vi "Create Channel.vi"(8 "error in (no error)":errorcluster, 10 "AIO_CFG":refnum<class "AIO-Configuration.lvclass">, 11 "UI Template in":refnum<class "AIO_Panel.lvclass">) -> (0 "error out":errorcluster, 3 "UI Template out":refnum<class "AIO_Panel.lvclass">)   [LabVIEW 2021, in "Simulator-Channel.lvlib" / "AIO_Panel.lvlib" / "AIO_Panel.lvclass"]
uses:
  AIO_Panel.lvclass
  Dependencies/AIO-Channel.lvlibp/Channels/AIO-Channel/AIO-Configuration_class/AIO-Configuration.lvclass
  C:/Users/averna/Documents/LV Gym DEMO/Factory Pattern/Device Channels/Dependencies/AIO-Channel.lvlibp/Generic Channel/Channel/Configuration_class/Configuration.lvclass
  tdef/info.ctl
  AIO_Panel.lvclass/AIO_Panel.ctl
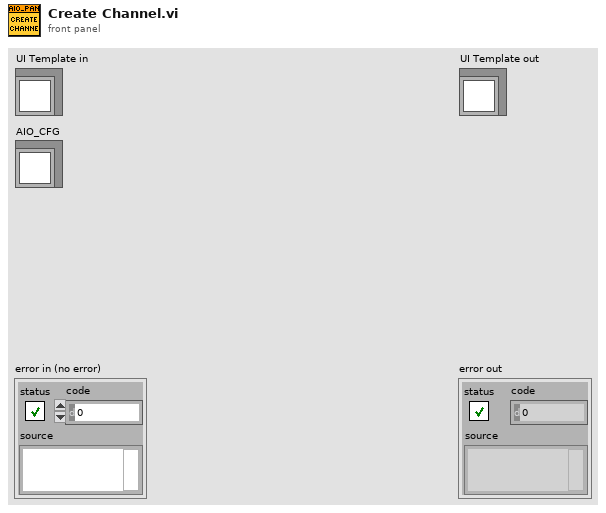
[diagram p1: front panel]
types:
  T1 = typedef "Simulator-Channel.lvlib/AIO_Panel.lvlib/AIO_Panel.lvclass/info.ctl" = cluster{"Name":string, "Numeric":dbl, "Unit":string}
  T2 = typedef "AIO-Channel.lvlibp/AIO-Configuration.lvclass/Direction.ctl" = enum16{"Input", "Output"}
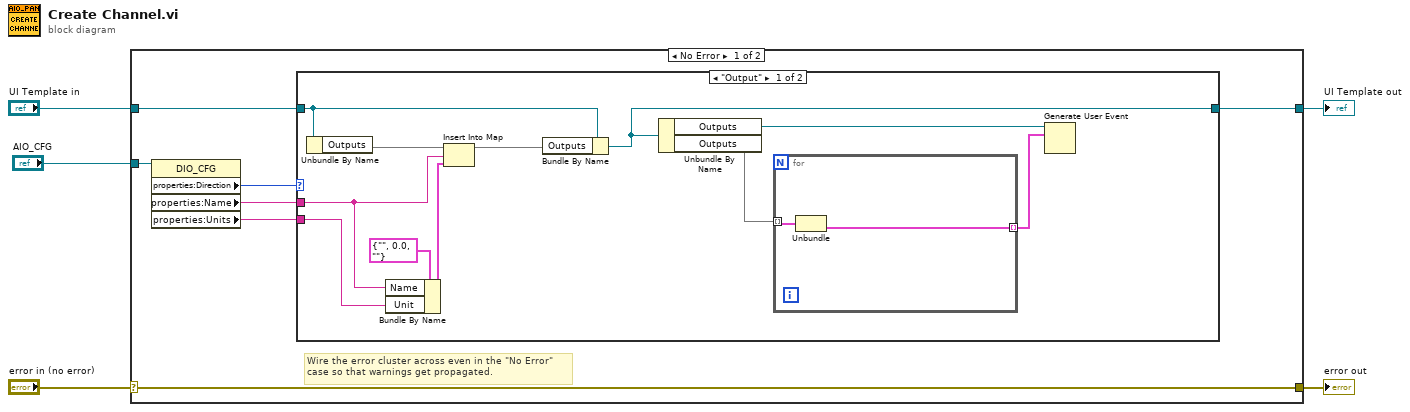
[diagram p0: block diagram]
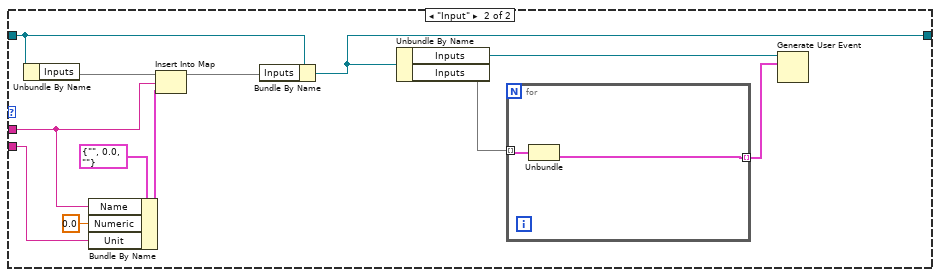
[diagram p2: hidden frame]
diagram:
  n1 = case shown="No Error" "error in (no error)" {
    selector: "error in (no error)" -> [w12 w41]
    tunnel: [w12 w41] -> w4
    tunnel: [w10 w40] -> w2
    tunnel: "UI Template in" -> [w9 w40]
    tunnel: "AIO_CFG" -> [w11 _]
    frame No Error {
      # "Wire the error cluster across even in the \"No Error\"\ncase so that warnings get propagated."
      n2 = property class="DIO_CFG"(reference=w11) -> ("properties:Direction"=w8:T2, "properties:Name"=w7:string, "properties:Units"=w6:string)  [unwired: 1 in, 2 out]
      n3 = case shown="\"Output\"" w8 {
        tunnel: [w18 w31] -> w10
        tunnel: w9 -> [w23 w37]
        tunnel: w7 -> [w14 w28]
        tunnel: w6 -> [w13 w27]
        frame "Output" {
          n4 = Unbundle By Name(w23) -> ("Outputs"=w22:map{string, T1})
          n5 = Bundle By Name(cluster=T1 {"Name"="", "Numeric"=0.0, "Unit"=""} ("value"), "Name"=w14, "Unit"=w13) -> (w15:T1)
          n6 = Insert Into Map(map in=w22, key=w14, value=w15) -> (map out=w21:map{string, T1})  [unwired: 2 out]
          n7 = Bundle By Name(cluster=w23, "Outputs"=w21) -> (w18:refnum<class "AIO_Panel.lvclass">)
          n8 = Unbundle By Name(w18) -> ("Outputs"=w19:refnum<user-event>, "Outputs"=w20:map{string, T1})
          n9 = for {
            tunnel: w20 -> [w25] mode=indexing
            tunnel: [w24] -> w17 mode=indexing
            n10 = Unbundle(w25) -> ("Info"=w24:T1)  [unwired: 1 out]
          }
          n11 = Generate User Event(user event=w19, event data cluster=w17) -> ()  [unwired: 2 in, 2 out]
        }
        frame "Input" {
          n12 = Unbundle By Name(w37) -> ("Inputs"=w36:map{string, T1})
          n13 = Bundle By Name(cluster=T1 {"Name"="", "Numeric"=0.0, "Unit"=""} ("value"), "Name"=w28, "Numeric"=0.0, "Unit"=w27) -> (w29:T1)
          n14 = Insert Into Map(map in=w36, key=w28, value=w29) -> (map out=w35:map{string, T1})  [unwired: 2 out]
          n15 = Bundle By Name(cluster=w37, "Inputs"=w35) -> (w31:refnum<class "AIO_Panel.lvclass">)
          n16 = Unbundle By Name(w31) -> ("Inputs"=w33:refnum<user-event>, "Inputs"=w34:map{string, T1})
          n17 = for {
            tunnel: w34 -> [w39] mode=indexing
            tunnel: [w38] -> w32 mode=indexing
            n18 = Unbundle(w39) -> ("Info"=w38:T1)  [unwired: 1 out]
          }
          n19 = Generate User Event(user event=w33, event data cluster=w32) -> ()  [unwired: 2 in, 2 out]
        }
      }
    }
    frame Error {
    }
  }
  "error out" <- w4
  "UI Template out" <- w2
